vi "Before Run TS.vi"(8 "error in":errorcluster, 11 "DeepU Test Stand in":refnum<class "DeepU Test Stand.lvclass">) -> (0 "error out":errorcluster, 3 "DeepU Test Stand out":refnum<class "DeepU Test Stand.lvclass">)   [LabVIEW 2019, in "Test Stands.lvlib" / "DeepU Test Stand.lvclass"]
uses:
  DeepU Test Stand.lvclass
  C:/Users/krio/Documents/LV_Projects/test-stand/App/Generic Test Stand/Generic Test Stand.lvclass
  DAC/DeepU/Inverter/DAC Inverter.lvclass
  C:/Users/krio/Documents/LV_Projects/test-stand/App/DAC/DAC.lvclass
  DAC/DeepU/FTCU/DAC FTCU.lvclass
  Generic Test Stand/Generic Test Stand.lvclass/Generic Test Stand.ctl
  DeepU Test Stand.lvclass/DeepU Test Stand.ctl
  DAC/DAC.lvclass/DAC.ctl
  DAC/DAC.lvclass
  Generic Test Stand/Generic Test Stand.lvclass
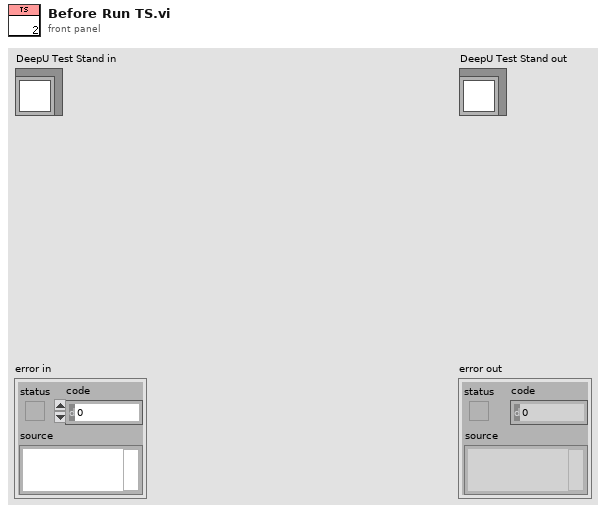
[diagram p1: front panel]
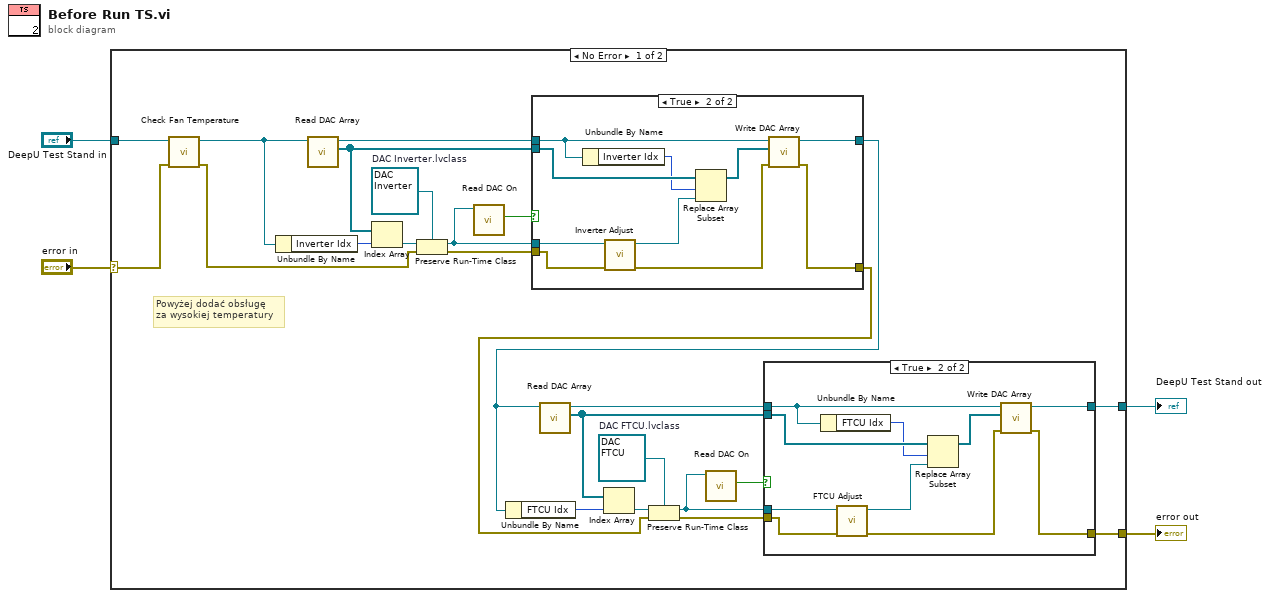
[diagram p0: block diagram]
diagram:
  n1 = case shown="No Error" "error in" {
    selector: "error in" -> [w6 w54]
    tunnel: [w10 w54] -> w1
    tunnel: [w11 w53] -> w2
    tunnel: "DeepU Test Stand in" -> [w8 w53]
    frame No Error {
      w9 = refnum<class "DAC FTCU.lvclass"> refnum  # DAC FTCU.lvclass
      w24 = refnum<class "DAC Inverter.lvclass"> refnum  # DAC Inverter.lvclass
      # "Powyżej dodać obsługę\nza wysokiej temperatury"
      n2 = call "Check Fan Temperature.vi"("error in"=w6, "DeepU Test Stand in"=w8) -> ("error out"=w5:errorcluster, "DeepU Test Stand out"=w7:refnum<class "DeepU Test Stand.lvclass">)  [unwired: 8 in]
      n3 = Unbundle By Name(w7) -> ("Inverter Idx"=w26:i32)
      n4 = call "Read DAC Array.vi"("Generic Test Stand in"=w7) -> ("DAC Array"=w21:refnum<class "DAC.lvclass">[], "Generic Test Stand out"=w27:refnum<class "DeepU Test Stand.lvclass">)  [unwired: 8 in, 1 out]
      n5 = Index Array(array=w21, index=w26) -> (element=w25:refnum<class "DAC.lvclass">)
      n6 = Preserve Run-Time Class(object in=w25, error in=w5, 2:w24) -> (object out=w23:refnum<class "DAC Inverter.lvclass">, error out=w22:errorcluster)
      n7 = call "Read DAC On.vi"("DAC in"=w23) -> ("DAC On"=w28:bool)  [unwired: 8 in, 2 out]
      n8 = case shown="True" w28 {
        tunnel: w27 -> [w42 w48]
        tunnel: [w42 w50] -> w14
        tunnel: w23 -> [_ w52]
        tunnel: w22 -> [w41 w51]
        tunnel: w21 -> [_ w49]
        tunnel: [w41 w43] -> w15
        frame False {
        }
        frame True {
          n9 = Unbundle By Name(w48) -> ("Inverter Idx"=w47:i32)
          n10 = call "Inverter Adjust.vi"("error in"=w51, "DAC Inverter in"=w52) -> ("error out"=w44:errorcluster, "DAC Inverter out"=w46:refnum<class "DAC Inverter.lvclass">)  [unwired: 8 in]
          n11 = Replace Array Subset(array=w49, new element=w46, index=w47) -> (w45:refnum<class "DAC.lvclass">[])
          n12 = call "Write DAC Array.vi"("error in (no error)"=w44, "DAC Array"=w45, "Generic Test Stand in"=w48) -> ("error out"=w43:errorcluster, "Generic Test Stand out"=w50:refnum<class "DeepU Test Stand.lvclass">)  [unwired: 7 in]
        }
      }
      n13 = Unbundle By Name(w14) -> ("FTCU Idx"=w17:i32)
      n14 = call "Read DAC Array.vi"("Generic Test Stand in"=w14) -> ("DAC Array"=w12:refnum<class "DAC.lvclass">[], "Generic Test Stand out"=w13:refnum<class "DeepU Test Stand.lvclass">)  [unwired: 8 in, 1 out]
      n15 = Index Array(array=w12, index=w17) -> (element=w18:refnum<class "DAC.lvclass">)
      n16 = Preserve Run-Time Class(object in=w18, error in=w15, 2:w9) -> (object out=w19:refnum<class "DAC FTCU.lvclass">, error out=w20:errorcluster)
      n17 = call "Read DAC On.vi"("DAC in"=w19) -> ("DAC On"=w16:bool)  [unwired: 8 in, 2 out]
      n18 = case shown="True" w16 {
        tunnel: w13 -> [w30 w36]
        tunnel: [w30 w38] -> w11
        tunnel: w19 -> [_ w40]
        tunnel: w20 -> [w29 w39]
        tunnel: w12 -> [_ w37]
        tunnel: [w29 w31] -> w10
        frame False {
        }
        frame True {
          n19 = Unbundle By Name(w36) -> ("FTCU Idx"=w35:i32)
          n20 = call "FTCU Adjust.vi"("error in"=w39, "DAC FTCU in"=w40) -> ("error out"=w32:errorcluster, "DAC FTCU out"=w34:refnum<class "DAC FTCU.lvclass">)  [unwired: 8 in]
          n21 = Replace Array Subset(array=w37, new element=w34, index=w35) -> (w33:refnum<class "DAC.lvclass">[])
          n22 = call "Write DAC Array.vi"("error in (no error)"=w32, "DAC Array"=w33, "Generic Test Stand in"=w36) -> ("error out"=w31:errorcluster, "Generic Test Stand out"=w38:refnum<class "DeepU Test Stand.lvclass">)  [unwired: 7 in]
        }
      }
    }
    frame Error {
    }
  }
  "error out" <- w1
  "DeepU Test Stand out" <- w2
